vi "startConsoleUi.vi"(8 "error in (no error)":errorcluster, 11 "Handler.UserEvent.Console in":refnum<class "Handler.UserEvent.Console.lvclass">) -> (0 "error out":errorcluster, 3 "Handler.UserEvent.Console out":refnum<class "Handler.UserEvent.Console.lvclass">)   [LabVIEW 2017, in "Error Log.lvlib" / "Handler.UserEvent.Console.lvclass"]
uses:
  Handler.UserEvent.Console.lvclass
  Handler.UserEvent.Console.lvclass/Handler.UserEvent.Console.ctl
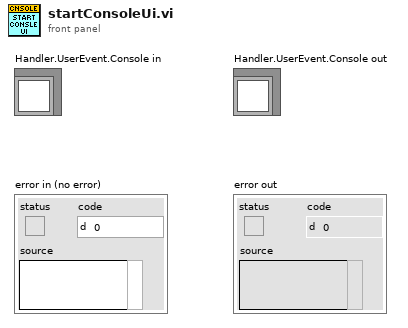
[diagram p1: front panel]
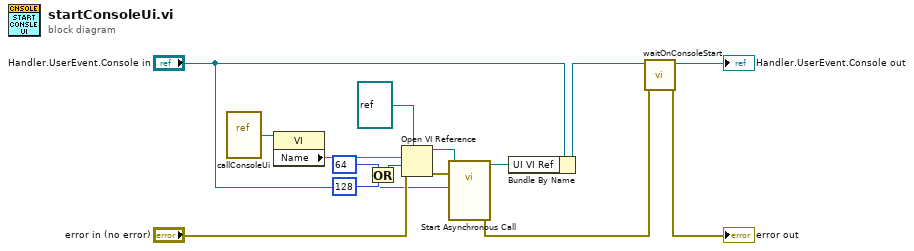
[diagram p0: block diagram]
diagram:
  n1 = vi-ref "callConsoleUi.vi"() -> (w15:refnum<vi>)
  n2 = property class="VI"(reference=w15) -> ("Name"=w14:string)  [unwired: 1 in, 2 out]
  n3 = Or(x=64, y=128 ("options")) -> (x .or. y?=w2:i32)
  n4 = Open VI Reference(type specifier VI Refnum (for type only)=refnum<vi> refnum, vi path=w14, options=w2, error in (no error)="error in (no error)") -> (vi reference=w13:refnum<vi>, error out=w10:errorcluster)  [unwired: 2 in]
  n5 = call-by-ref "Start Asynchronous Call"(reference=w13, error in=w10, "Handler.UserEvent.Console in"="Handler.UserEvent.Console in") -> (reference out=w7:refnum<vi>, error out=w4:errorcluster)  [unwired: 9 in, 2 out]
  n6 = Bundle By Name(cluster="Handler.UserEvent.Console in", "UI VI Ref"=w7) -> (w6:refnum<class "Handler.UserEvent.Console.lvclass">)
  n7 = call "waitOnConsoleStart.vi"("error in (no error)"=w4, "Handler.UserEvent.Console in"=w6) -> ("error out"=→"error out":errorcluster, "Handler.UserEvent.Console out"=→"Handler.UserEvent.Console out":refnum<class "Handler.UserEvent.Console.lvclass">)  [unwired: 8 in]
